vi "graph display.vi"(9 "Graph Type":u16, 10 "DATA":dbl[][](array[numeric]), 11 "XYGraph in":refnum<vi>) -> (3 "Array":cluster{"DATA":dbl[], "DATA":dbl[]}[](array[cluster]))   [LabVIEW 2026]
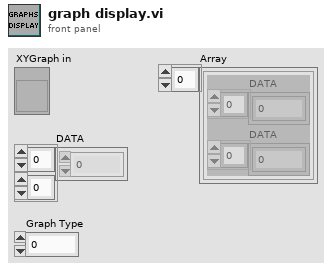
[diagram p1: front panel]
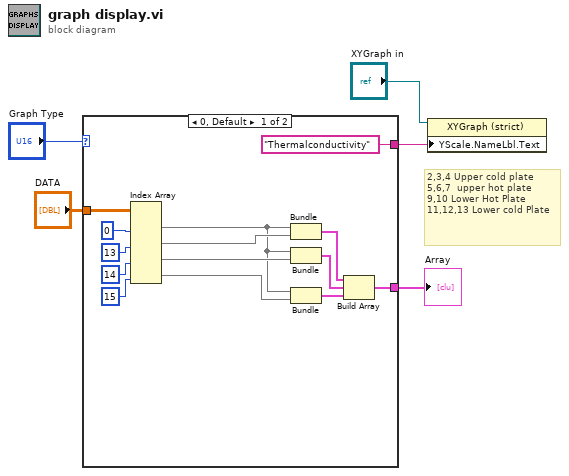
[diagram p0: block diagram]
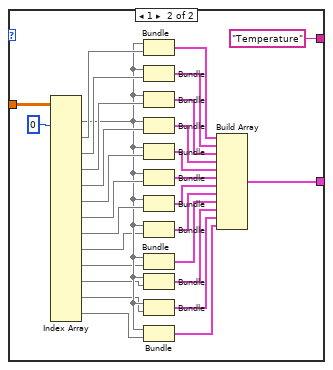
[diagram p2: hidden frame]
diagram:
  # "2,3,4 Upper cold plate\n5,6,7  upper hot plate\n9,10 Lower Hot Plate\n11,12,13 Lower cold Plate"
  n1 = case shown="0, Default" "Graph Type" {
    tunnel: "DATA" -> [w19 w48]
    tunnel: [w16 w22] -> w3
    tunnel: ["Thermalconductivity" "Temperature"] -> w4
    frame 0, Default {
      n2 = Index Array(array=w19, index (col) #1=0 ("disabled index (col)"), index (col) #2=13 ("index (col)"), index (col) #3=14 ("index (col)"), index (col) #4=15 ("index (col)")) -> (element #1=w9:dbl[], element #2=w18:dbl[], element #3=w13:dbl[], element #4=w12:dbl[])  [unwired: 4 in]
      n3 = Bundle("DATA"=w9, "DATA"=w18) -> (w17:cluster{"DATA":dbl[], "DATA":dbl[]})  [unwired: 1 in]
      n4 = Bundle("DATA"=w9, "DATA"=w13) -> (w11:cluster{"DATA":dbl[], "DATA":dbl[]})  [unwired: 1 in]
      n5 = Bundle("DATA"=w9, "DATA"=w12) -> (w10:cluster{"DATA":dbl[], "DATA":dbl[]})  [unwired: 1 in]
      n6 = Build Array(w17, w11, w10) -> (w16:cluster{"DATA":dbl[], "DATA":dbl[]}[])
    }
    frame 1 {
      n7 = Index Array(array=w48, index (col) #1=0 ("disabled index (col)")) -> (element #1=w39:dbl[], element #2=w47:dbl[], element #3=w45:dbl[], element #4=w44:dbl[], element #5=w43:dbl[], element #6=w42:dbl[], element #7=w41:dbl[], element #8=w40:dbl[], element #9=w38:dbl[], element #10=w37:dbl[], element #11=w36:dbl[], element #12=w35:dbl[], element #13=w34:dbl[])  [unwired: 25 in]
      n8 = Bundle("DATA"=w39, "DATA"=w47) -> (w46:cluster{"DATA":dbl[], "DATA":dbl[]})  [unwired: 1 in]
      n9 = Bundle("DATA"=w39, "DATA"=w45) -> (w33:cluster{"DATA":dbl[], "DATA":dbl[]})  [unwired: 1 in]
      n10 = Bundle("DATA"=w39, "DATA"=w44) -> (w32:cluster{"DATA":dbl[], "DATA":dbl[]})  [unwired: 1 in]
      n11 = Bundle("DATA"=w39, "DATA"=w43) -> (w31:cluster{"DATA":dbl[], "DATA":dbl[]})  [unwired: 1 in]
      n12 = Bundle("DATA"=w39, "DATA"=w42) -> (w30:cluster{"DATA":dbl[], "DATA":dbl[]})  [unwired: 1 in]
      n13 = Bundle("DATA"=w39, "DATA"=w41) -> (w29:cluster{"DATA":dbl[], "DATA":dbl[]})  [unwired: 1 in]
      n14 = Bundle("DATA"=w39, "DATA"=w40) -> (w28:cluster{"DATA":dbl[], "DATA":dbl[]})  [unwired: 1 in]
      n15 = Bundle("DATA"=w39, "DATA"=w38) -> (w27:cluster{"DATA":dbl[], "DATA":dbl[]})  [unwired: 1 in]
      n16 = Bundle("DATA"=w39, "DATA"=w37) -> (w26:cluster{"DATA":dbl[], "DATA":dbl[]})  [unwired: 1 in]
      n17 = Bundle("DATA"=w39, "DATA"=w36) -> (w25:cluster{"DATA":dbl[], "DATA":dbl[]})  [unwired: 1 in]
      n18 = Bundle("DATA"=w39, "DATA"=w35) -> (w24:cluster{"DATA":dbl[], "DATA":dbl[]})  [unwired: 1 in]
      n19 = Bundle("DATA"=w39, "DATA"=w34) -> (w23:cluster{"DATA":dbl[], "DATA":dbl[]})  [unwired: 1 in]
      n20 = Build Array(w46, w33, w32, w31, w30, w29, w28, w27, w26, w25, w24, w23) -> (w22:cluster{"DATA":dbl[], "DATA":dbl[]}[])
    }
  }
  "Array" <- w3
  n21 = property on="Property Node" class="XYGraph (strict)"(reference="XYGraph in", "YScale.NameLbl.Text"=w4) -> ()  [unwired: 1 in, 2 out]
